vi "query Call Processing Status.vi"(8 "error in (no error)":errorcluster, 11 "Anritsu Call Box in":refnum<class "Anritsu Call Box.lvclass">) -> (0 "error out":errorcluster, 2 "Call Processing Status":T1, 3 "Anritsu Call Box out":refnum<class "Anritsu Call Box.lvclass">)   [LabVIEW 2023, in "ANRITSU Call Box.lvlib" / "Anritsu Call Box.lvclass"]
doc: "Call Processing Status는 NR / LTE 동일."
uses:
  Anritsu Call Box.lvclass
  Type Definition/Call Processing Status Enum.ctl
  ANRITSU Call Box.lvlib
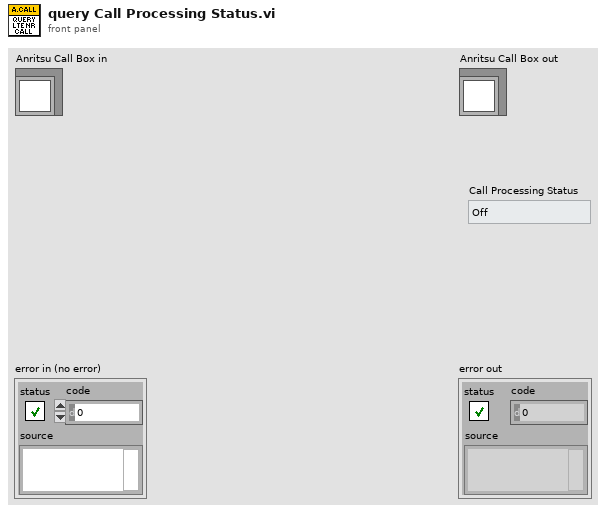
[diagram p1: front panel]
types:
  T1 = typedef "ANRITSU Call Box.lvlib/Call Processing Status Enum.ctl" = enum16{"Off", "Idle", "Idle (Regist)", "Registration", "UE Origination", "NW Origination", "Connected", "SCG Adding", "Connected (NSA)", "SCG Release", "Undefined1", "Undefined2", "Undefined3", "Handover", "NW Release", "UE Release", "Detach", "Setup", "Redirection"}
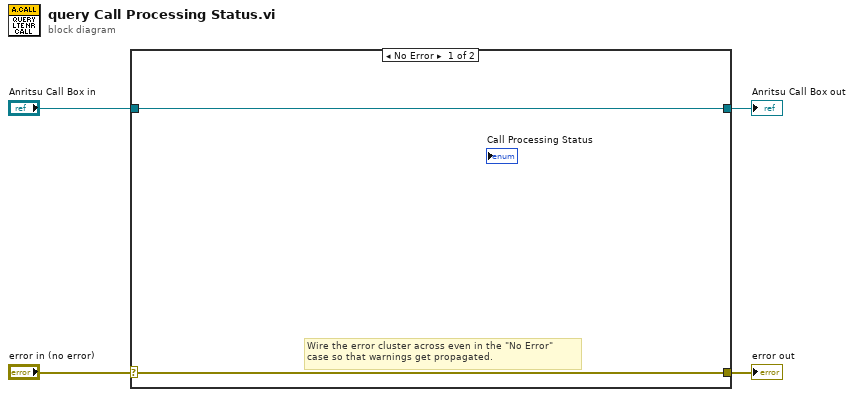
[diagram p0: block diagram]
diagram:
  n1 = case shown="No Error" "error in (no error)" {
    selector: "error in (no error)" -> [w5 w8]
    tunnel: [w5 w8] -> w3
    tunnel: [w6 w7] -> w1
    tunnel: "Anritsu Call Box in" -> [w6 w7]
    frame No Error {
      # "Wire the error cluster across even in the \"No Error\"\ncase so that warnings get propagated."
    }
    frame Error {
    }
  }
  "error out" <- w3
  "Anritsu Call Box out" <- w1
